vi "Serial no Read & Write.vi"(8 "error in":errorcluster, 11 "PCB Serial No":string) -> (0 "error out":errorcluster, 1 "Command Response":string, 2 "Result":string, 3 "RESULT":bool)   [LabVIEW 2021]
uses:
  10054_Control Folder/Support/Relay_no.ctl
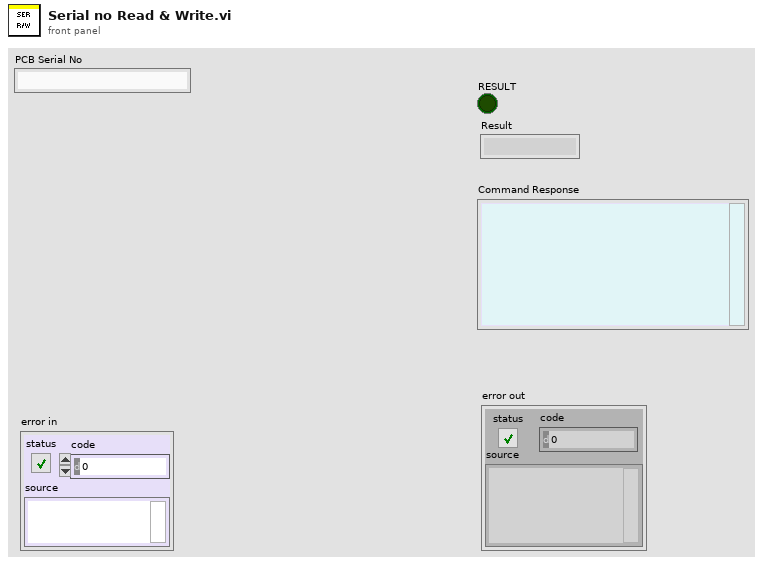
[diagram p1: front panel]
types:
  T1 = typedef "Relay_no.ctl" = enum16{"Init", "write&Read", "PCB Serial Write & Read", "PCB Write SSD & Password", "Read Wifi state", "Reset", "Close"}
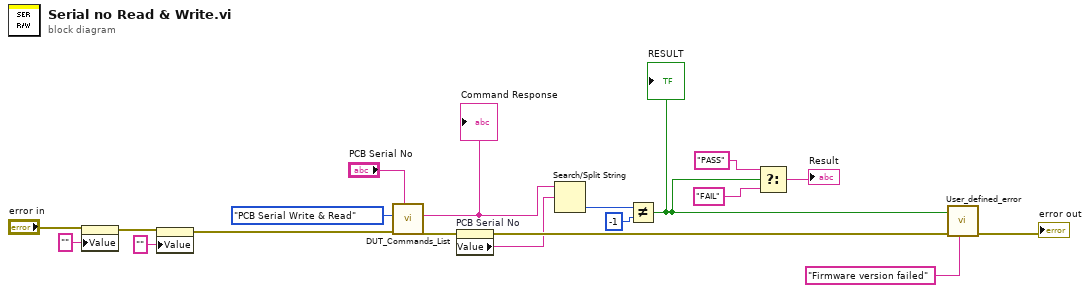
[diagram p0: block diagram]
diagram:
  n1 = property on="PCB Serial No" class="Str"(error in="error in", "Value"="" ("PCB Serial No")) -> (error out=w1:errorcluster)  [unwired: 1 in, 1 out]
  n2 = property on="Command Response" class="Str"(error in=w1, "Value"="" ("Command Response")) -> (error out=w10:errorcluster)  [unwired: 1 in, 1 out]
  n3 = call "DUT_Commands_List.vi"("PCB Serial No"="PCB Serial No", "error in"=w10, "Operation"=Relay_no."PCB Serial Write & Read") -> ("error out"=w6:errorcluster, "Command Response"=w11:string)  [unwired: 6 in, 1 out]
  "Command Response" <- w11
  n4 = property on="PCB Serial No" class="Str"(error in=w6) -> (error out=w5:errorcluster, "Value"=w4:string)  [unwired: 1 in, 1 out]
  n5 = Search/Split String(string=w11, search string/char (-)=w4) -> (offset of match=w18:i32)  [unwired: 1 in, 2 out]
  n6 = Not Equal?(x=w18, y=-1) -> (x != y?=w15:bool)
  "RESULT" <- w15
  n7 = Select(t="PASS", s=w15, f="FAIL") -> (s? t:f=→"Result":string)
  n8 = call "User_defined_error.vi"("Error Msg"="Firmware version failed" ("source"), "error in"=w5, "Result"=w15) -> ("error Out"=→"error out":errorcluster)  [unwired: 8 in]
